vi "test notification accepted.vi"(8 "error in (no error)":errorcluster) -> (0 "error out":errorcluster, 3 "body":string)   [LabVIEW 2020, in "MCP Server tests.lvlib"]
doc: "A notification (a message without id) must be answered with 202 Accepted and an empty body."
uses:
  MCP Server tests.lvlib
  <vilib>/addons/_JKI Toolkits/Caraya/classes/Test/Test.lvclass
  <vilib>/addons/_JKI Toolkits/Caraya/classes/Assert/Assert.lvclass
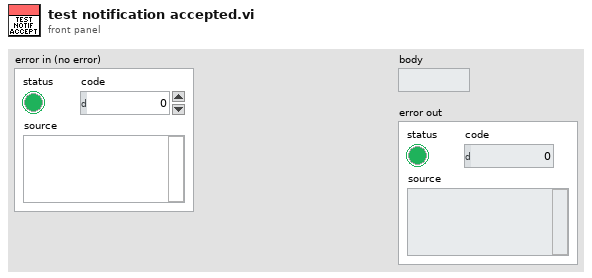
[diagram p1: front panel]
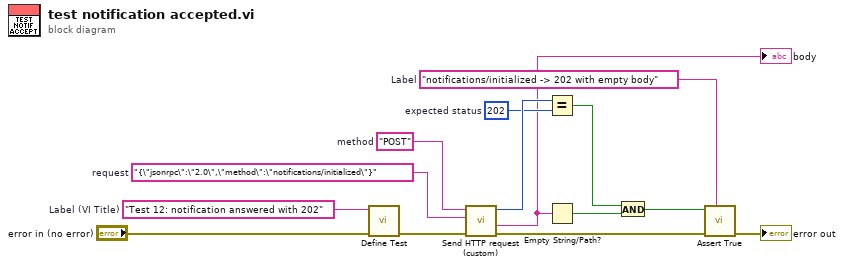
[diagram p0: block diagram]
diagram:
  w3 = "notifications/initialized -> 202 with empty body"  # Label
  w8 = 202  # expected status
  w11 = "{\"jsonrpc\":\"2.0\",\"method\":\"notifications/initialized\"}"  # request
  w12 = "POST"  # method
  w14 = "Test 12: notification answered with 202"  # Label (VI Title)
  n1 = call <vilib>:"Define Test.vi"("error in (no error)"="error in (no error)", "Label (VI Title)"=w14) -> ("error out"=w10:errorcluster)  [unwired: 8 in, 1 out]
  n2 = call "Send HTTP request (custom).vi"("error in (no error)"=w10, "request"=w11, "method"=w12) -> ("error out"=w4:errorcluster, "response"=w2:string, "status code"=w9:i32)  [unwired: 5 in, 1 out]
  "body" <- w2
  n3 = Equal?(x=w9, y=w8) -> (x = y?=w7:bool)
  n4 = Empty String/Path?(string/path=w2) -> (empty?=w6:bool)
  n5 = And(x=w7, y=w6) -> (x .and. y?=w5:bool)
  n6 = call <vilib>:"Assert True.vi"("Label"=w3, "error in (no error)"=w4, "True?"=w5) -> ("error out"=→"error out":errorcluster)  [unwired: 7 in, 1 out]
